vi "onDestroyDebugTerminal.vi"(8 "error in (no error)":errorcluster, 11 "DebuggingTerminal in":refnum<class "DebuggingTerminal.lvclass">) -> (0 "error out":errorcluster, 3 "DebuggingTerminal out":refnum<class "DebuggingTerminal.lvclass">)   [LabVIEW 2013, in "MQTT Base.lvlib" / "DebuggingTerminal.lvclass"]
uses:
  DebuggingTerminal.lvclass
  DebuggingTerminal.lvclass/DebuggingTerminal.ctl
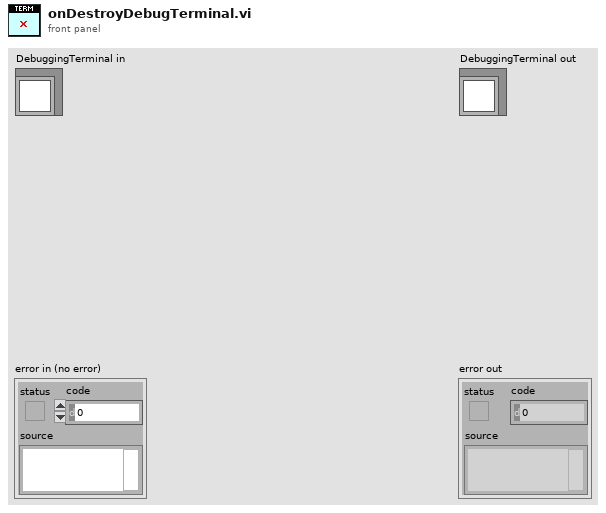
[diagram p1: front panel]
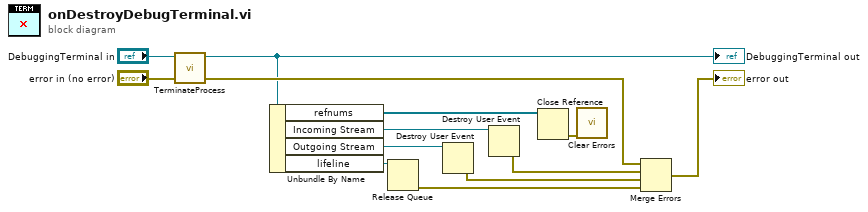
[diagram p0: block diagram]
diagram:
  n1 = call "TerminateProcess.vi"("DebuggingTerminal in"="DebuggingTerminal in") -> ("DebuggingTerminal out"=w3:refnum<class "DebuggingTerminal.lvclass">)  [unwired: 10 in]
  "DebuggingTerminal out" <- w3
  n2 = Unbundle By Name(w3) -> ("refnums"=w2:refnum<vi>[], "Incoming Stream"=w12:refnum<user-event>, "Outgoing Stream"=w11:refnum<user-event>, "lifeline"=w5:refnum<queue>)
  n3 = Release Queue(queue=w5) -> (error out=w8:errorcluster)  [unwired: 2 in, 2 out]
  n4 = Destroy User Event(user event=w11) -> (error out=w7:errorcluster)  [unwired: 1 in]
  n5 = Destroy User Event(user event=w12) -> (error out=w6:errorcluster)  [unwired: 1 in]
  n6 = Close Reference(reference=w2) -> (error out=w1:errorcluster)  [unwired: 1 in]
  n7 = call <vilib>:"Clear Errors.vi"("error in (no error)"=w1) -> ()  [unwired: 6 in, 1 out]
  n8 = Merge Errors("error in (no error)", w6, w7, w8) -> (→"error out":errorcluster)
